vi "GetTerms3.vi"(0 "XRef":T10, 1 "State In":T9) -> (14 "Terms":T1)   [LabVIEW 2012, in "OpenG Index Array Element.xnode"]
doc: "This ability VI is used to describe your terminals to LabVIEW. Terms is an array of clusters describing the XNode's terminals.\n ID: A unique string identifying the terminal.\n Name: The name of the terminal visible to the user. Remember to localize it.\n Type: The data type of the terminal (as a Variant). The data put in the variant will be used as the default for the input terminal if it's left unwired.\n Bounds: A rectangle defining the bounds of the terminal relative to the bounds of the XNode. The bounds must be within the bounds of the XNode, and for whiskers to draw properly, they must be flush with at least one side of the XNode.\n Input?: Indicates whether or not this terminals is an input.\n Required?: Indicates whether the user must wire this terminal for the XNode to not be broken. Ignored on outputs.\n Recommended?: Indicates whether the terminal is recommended.\n Hidden?: Indicates whether the terminal is hidden. When a terminal is hidden, it cannot be wired to via user interaction or scripting. However, if it is already wired to when the hidden flag is changed to true, it will remain wired.\n Adaptive?: Indicates that the term should change to match the type of its source if it is wired.\n Direction?: Indicates what direction the wire stub should point. Choose auto to let LV decide based on the terms bounds being on the nodes edge.\n \n The IDs are used by LabVIEW to keep track of your terminals. When you respecify your terminals, LabVIEW can tell whther terminals are new, deleted, or moved by the unique IDs. The order is irrelevant. If you move a terminal, then any wire connected to it will move with it.\n \n If you want to update your terminals, you should return the UpdateTerms reply in one of your ability VIs.\n\nDefault behavior: None.\n\nThis ability does not provide UI and OS messages are not handled."
uses:
  OpenG Index Array Element.xnode
  <vilib>/XNodeSupport/XNodeXNodeRef.ctl
  State.ctl
  <vilib>/XNodeSupport/XNodeTerm3Array.ctl
  <vilib>/XNodeSupport/XNodeTerm3.ctl
  <vilib>/XNodeSupport/XNodeString.ctl
  <vilib>/XNodeSupport/XNodeVariant.ctl
  <vilib>/XNodeSupport/XNodeRect32.ctl
  <vilib>/XNodeSupport/XNodeInt.ctl
  <vilib>/XNodeSupport/XNodeBool.ctl
  <vilib>/XNodeSupport/XNodeTermDirection.ctl
  <vilib>/XNodeSupport/NI_XNodeSupport.lvlib
  <vilib>/Utility/VariantDataType/VariantType.lvlib
  VI Scripting/Scripting Tools/XNode Support/XNode Support.lvlib
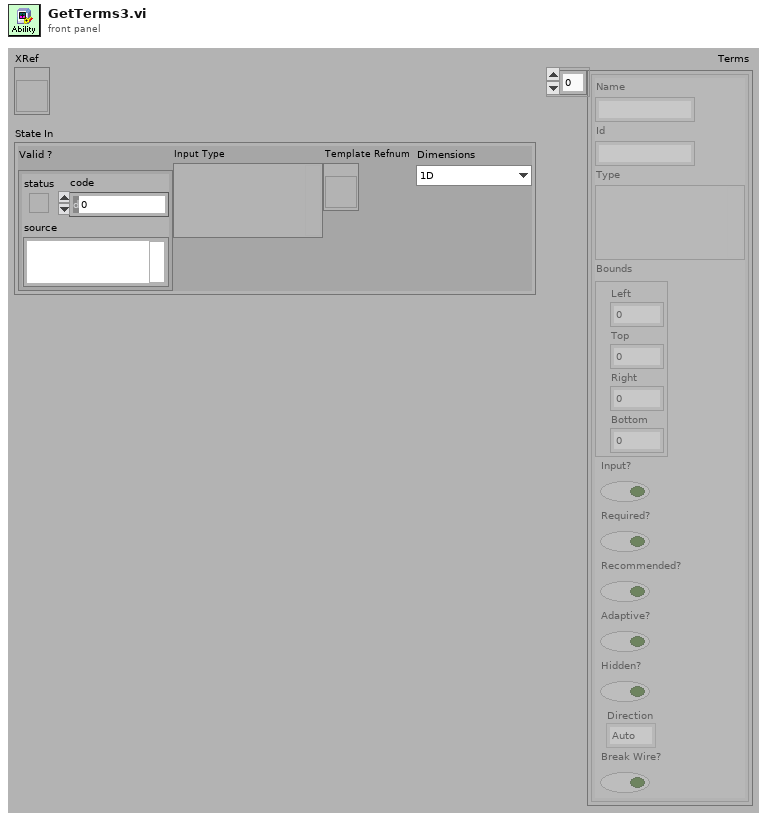
[diagram p1: front panel]
types:
  T1 = typedef "NI_XNodeSupport.lvlib/XNodeTerm3Array.ctl" = T2[]
  T2 = typedef "NI_XNodeSupport.lvlib/XNodeTerm3.ctl" = cluster{"Name":T3, "Id":T3, "Type":T4, "Bounds":T5, "Input?":T7, "Required?":T7, "Recommended?":T7, "Adaptive?":T7, "Hidden?":T7, "Direction":T8, "Break Wire?":T7}
  T3 = typedef "NI_XNodeSupport.lvlib/XNodeString.ctl" = string
  T4 = typedef "NI_XNodeSupport.lvlib/XNodeVariant.ctl" = variant
  T5 = typedef "NI_XNodeSupport.lvlib/XNodeRect32.ctl" = cluster{"Left":T6, "Top":T6, "Right":T6, "Bottom":T6}
  T6 = typedef "NI_XNodeSupport.lvlib/XNodeInt.ctl" = i32
  T7 = typedef "NI_XNodeSupport.lvlib/XNodeBool.ctl" = bool
  T8 = typedef "NI_XNodeSupport.lvlib/XNodeTermDirection.ctl" = enum32{"Auto", "Up", "Down", "Left", "Right", "Center"}
  T9 = typedef "OpenG Index Array Element.xnode/State.ctl" = cluster{"Valid ?":errorcluster, "Input Type":variant, "Template Refnum":refnum<vi>, "Dimensions":enum16{"1D", "2D"}}
  T10 = typedef "NI_XNodeSupport.lvlib/XNodeXNodeRef.ctl" = refnum<vi>
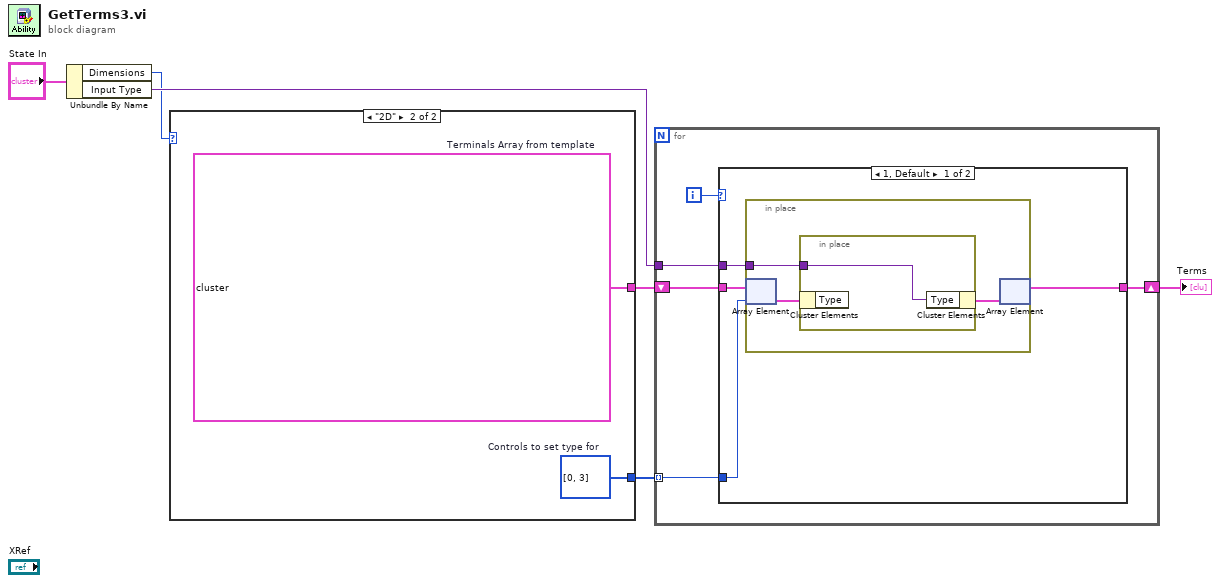
[diagram p0: block diagram]
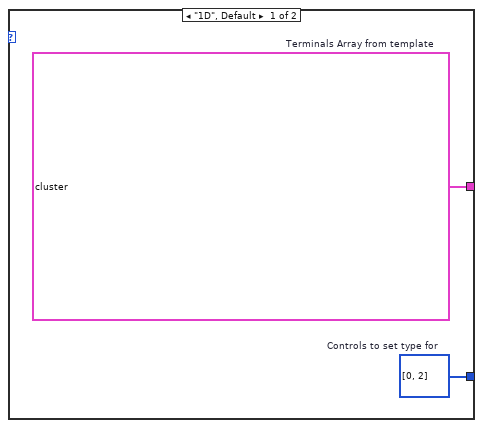
[diagram p2: hidden frame]
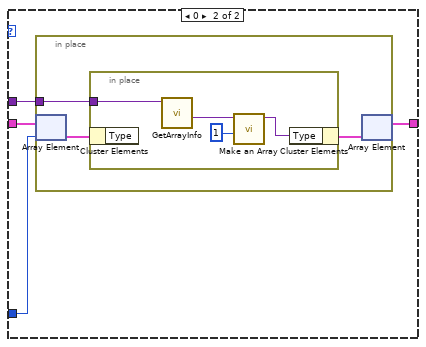
[diagram p3: hidden frame]
diagram:
  n1 = Unbundle By Name("State In") -> ("Dimensions"=w1:enum16{"1D", "2D"}, "Input Type"=w6:variant)
  n2 = case shown="\"2D\"" w1 {
    tunnel: [w8 w10] -> w5
    tunnel: [w7 w9] -> w4
    frame "1D", Default {
      w7 = i32[] [0, 2]  # Controls to set type for
      w8 = T2[] [{"Name"="elements", "Id"="1", "Type"=variant(dbl[] []), "Bounds"={"Left"=24, "Top"=16, "Right"=32, "Bottom"=24}, "Input?"=FALSE, "Required?"=FALSE, "Recommended?"=TRUE, "Adaptive?"=FALSE, "Hidden?"=FALSE, "Direction"=enum."Auto", "Break Wire?"=FALSE}, {"Name"="indices", "Id"="9", "Type"=variant(i32[] []), "Bounds"={"Left"=0, "Top"=16, "Right"=8, "Bottom"=24}, "Input?"=TRUE, "Required?"=TRUE, "Recommended?"=TRUE, "Adaptive?"=FALSE, "Hidden?"=FALSE, "Direction"=enum."Auto", "Break Wire?"=FALSE}, {"Name"="array", "Id"="11", "Type"=variant(dbl[] []), "Bounds"={"Left"=0, "Top"=0, "Right"=8, "Bottom"=8}, "Input?"=TRUE, "Required?"=TRUE, "Recommended?"=TRUE, "Adaptive?"=FALSE, "Hidden?"=FALSE, "Direction"=enum."Auto", "Break Wire?"=FALSE}]  # Terminals Array from template
    }
    frame "2D" {
      w9 = i32[] [0, 3]  # Controls to set type for
      w10 = T2[] [{"Name"="elements", "Id"="1", "Type"=variant(dbl[] []), "Bounds"={"Left"=24, "Top"=16, "Right"=32, "Bottom"=24}, "Input?"=FALSE, "Required?"=FALSE, "Recommended?"=TRUE, "Adaptive?"=FALSE, "Hidden?"=FALSE, "Direction"=enum."Auto", "Break Wire?"=FALSE}, {"Name"="indices 1", "Id"="8", "Type"=variant(i32[] []), "Bounds"={"Left"=0, "Top"=24, "Right"=8, "Bottom"=32}, "Input?"=TRUE, "Required?"=TRUE, "Recommended?"=TRUE, "Adaptive?"=FALSE, "Hidden?"=FALSE, "Direction"=enum."Auto", "Break Wire?"=FALSE}, {"Name"="indices 0", "Id"="9", "Type"=variant(i32[] []), "Bounds"={"Left"=0, "Top"=16, "Right"=8, "Bottom"=24}, "Input?"=TRUE, "Required?"=TRUE, "Recommended?"=TRUE, "Adaptive?"=FALSE, "Hidden?"=FALSE, "Direction"=enum."Auto", "Break Wire?"=FALSE}, {"Name"="array", "Id"="11", "Type"=variant(dbl[][] []), "Bounds"={"Left"=0, "Top"=0, "Right"=8, "Bottom"=8}, "Input?"=TRUE, "Required?"=TRUE, "Recommended?"=TRUE, "Adaptive?"=FALSE, "Hidden?"=FALSE, "Direction"=enum."Auto", "Break Wire?"=FALSE}]  # Terminals Array from template
    }
  }
  n3 = for {
    tunnel: w6 -> [w14]
    shift-right: [w13] -> w3
    shift-left: w5 -> [w15]
    tunnel: w4 -> [w12] mode=indexing
    i -> [w11]
    n4 = case shown="1, Default" w11 {
      tunnel: w15 -> [w19 w27]
      tunnel: w14 -> [w18 w26]
      tunnel: [w17 w25] -> w13
      tunnel: w12 -> [w16 w24]
      frame 1, Default {
        n5 = in-place {
          in-place-border: w18 -> [w21]
          n6 = in-place-array #1(w19, w16) -> (w22:T2)
          n7 = in-place {
            in-place-border: w21 -> [w23]
            n8 = in-place-cluster #2(w22) -> ()  [unwired: 1 out]
            n9 = in-place-cluster #2("Type"=w23) -> (w20:T2)
          }
          n10 = in-place-array #1(w20) -> (w17:T2[])  [unwired: 1 out]
        }
      }
      frame 0 {
        n11 = in-place {
          in-place-border: w26 -> [w29]
          n12 = in-place-array #3(w27, w24) -> (w30:T2)
          n13 = in-place {
            in-place-border: w29 -> [w34]
            n14 = in-place-cluster #4(w30) -> ()  [unwired: 1 out]
            n15 = call <vilib>:"GetArrayInfo.vi"("Variant"=w34) -> ("ArrayElement"=w33:variant)  [unwired: 1 in, 9 out]
            n16 = call <userlib>:"Make an Array.vi"("Number of Dimensions"=1, "Element Type"=w33) -> ("Array Type"=w31:variant)  [unwired: 1 in, 8 out]
            n17 = in-place-cluster #4("Type"=w31) -> (w28:T2)
          }
          n18 = in-place-array #3(w28) -> (w25:T2[])  [unwired: 1 out]
        }
      }
    }
  }
  "Terms" <- w3
